vi "Connect.vi"(8 "error in (no error)":errorcluster, 11 "object in":refnum<class "AIO_Channel.lvclass">) -> (0 "error out":errorcluster, 2 "Success?":bool, 3 "object out":refnum<class "AIO_Channel.lvclass">)   [LabVIEW 2021, in "Simulator-Channel.lvlib" / "AIO_Channel.lvclass"]
uses:
  AIO_Channel.lvclass
  C:/Users/averna/Documents/LV Gym DEMO/Factory Pattern/Device Channels/Dependencies/AIO-Channel.lvlibp/Channels/AIO-Channel/AIO_Channel_class/AIO_Channel.lvclass
  AIO_Panel/DIO_Panel Messages/Create Channel Msg/Create Channel Msg.lvclass/Create Channel Msg.ctl
  <vilib>/ActorFramework/Message Enqueuer/Message Enqueuer.lvclass/Message Enqueuer.ctl
  AIO_Channel.lvclass/AIO_Channel.ctl
  <vilib>/ActorFramework/Message Enqueuer/Enqueue.vi
  AIO_Panel/DIO_Panel Messages/Create Channel Msg/Create Channel Msg.lvclass
  C:/Program Files/National Instruments/LabVIEW 2021/vi.lib/ActorFramework/Message/Message.lvclass
  Dependencies/AIO-Channel.lvlibp/Channels/AIO-Channel/AIO_Channel_class/Properties/GetAIOConfiguration.vi
  <vilib>/ActorFramework/Message Priority Queue/Priority Enqueue.vi
  Dependencies/AIO-Channel.lvlibp/Channels/AIO-Channel/AIO-Configuration_class/AIO-Configuration.lvclass
  Simulator-Channel.lvlib
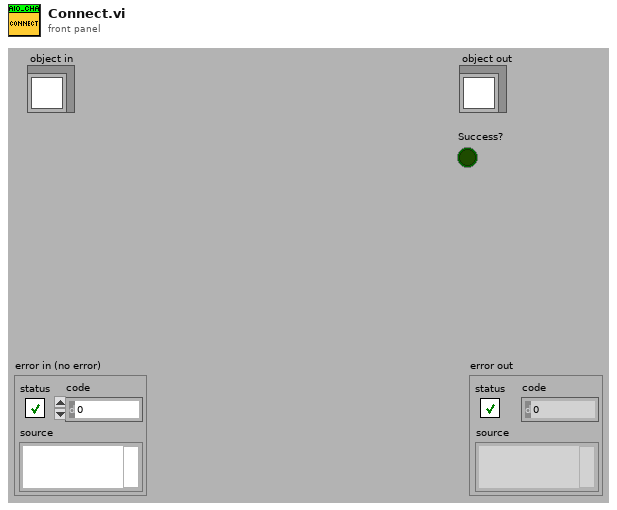
[diagram p1: front panel]
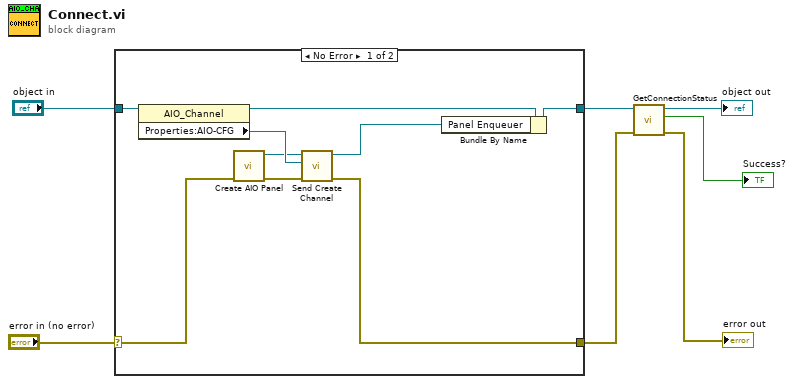
[diagram p0: block diagram]
diagram:
  n1 = case shown="No Error" "error in (no error)" {
    selector: "error in (no error)" -> [w15 w18]
    tunnel: [w12 w18] -> w3
    tunnel: [w14 w17] -> w5
    tunnel: "object in" -> [w16 w17]
    frame No Error {
      n2 = property class="AIO_Channel"(reference=w16) -> (reference out=w11:refnum<class "AIO_Channel.lvclass">, "Properties:AIO-CFG"=w10:refnum<class "AIO-Configuration.lvclass">)  [unwired: 1 in, 1 out]
      n3 = call "Create AIO Panel.vi"("error in (no error)"=w15) -> ("error out"=w13:errorcluster, "Panel Enqueuer"=w9:refnum<class "Message Enqueuer.lvclass">)  [unwired: 9 in]
      n4 = call "Send Create Channel.vi"("error in (no error)"=w13, "AIO_CFG"=w10, "Message Enqueuer"=w9) -> ("error out"=w12:errorcluster, "Message Enqueuer out"=w8:refnum<class "Message Enqueuer.lvclass">)  [unwired: 7 in]
      n5 = Bundle By Name(cluster=w11, "Panel Enqueuer"=w8) -> (w14:refnum<class "AIO_Channel.lvclass">)
    }
    frame Error {
    }
  }
  n6 = call-dynamic "GetConnectionStatus.vi"("error in (no error)"=w3, "object in"=w5) -> ("error out"=→"error out":errorcluster, "Connected?"=→"Success?":bool, "object out"=→"object out":refnum<class "AIO_Channel.lvclass">)  [unwired: 7 in]
